vi "GetStopEvent.vi"(8 "error in (no error)":errorcluster, 11 "NavigatableView in":refnum<class "NavigatableView.lvclass">) -> (0 "error out":errorcluster, 2 "StopEvent":refnum<user-event>, 3 "NavigatableView out":refnum<class "NavigatableView.lvclass">)   [LabVIEW 2024, in "NavigatableView.lvclass"]
doc: "Return stop event for view to register."
uses:
  NavigatableView.lvclass
  NavigatableView.lvclass/NavigatableView.ctl
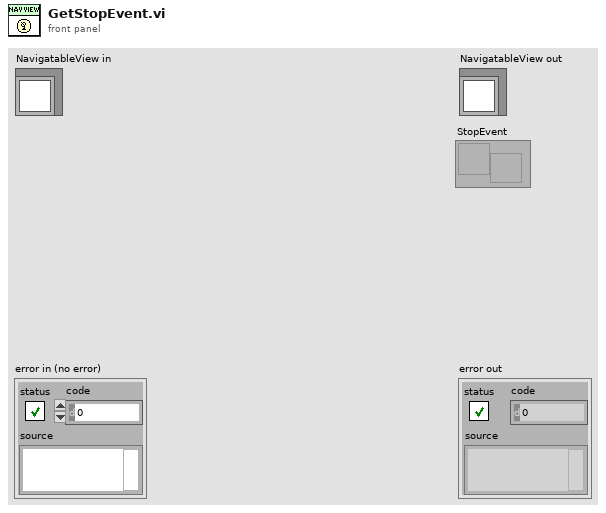
[diagram p1: front panel]
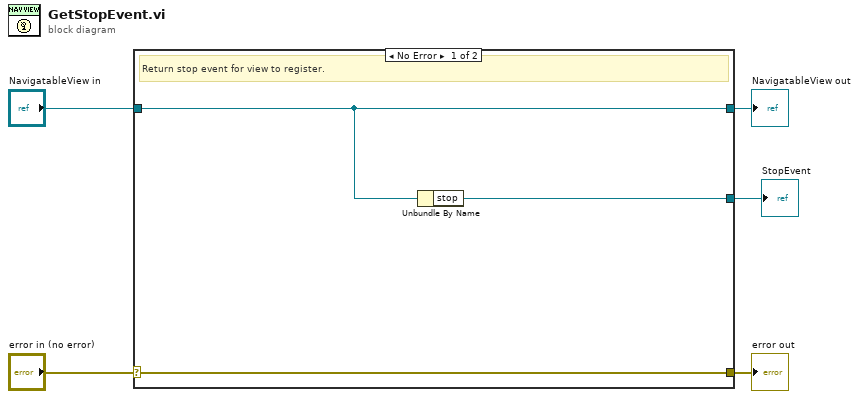
[diagram p0: block diagram]
diagram:
  n1 = case shown="No Error" "error in (no error)" {
    selector: "error in (no error)" -> [w8 w10]
    tunnel: [w8 w10] -> w4
    tunnel: [w7 w9] -> w2
    tunnel: "NavigatableView in" -> [w7 w9]
    tunnel: [w6 _] -> w1
    frame No Error {
      # "Return stop event for view to register."
      n2 = Unbundle By Name(w7) -> ("stop"=w6:refnum<user-event>)
    }
    frame Error {
    }
  }
  "error out" <- w4
  "NavigatableView out" <- w2
  "StopEvent" <- w1
